vi "NR set BandWidth.vi"(8 "error in (no error)":errorcluster caption="에러 입력(에러 없음)", 10 "BW (MHz)":u32, 11 "Instrument Manager 입력":refnum<class "Instrument Manager.lvclass">) -> (0 "error out":errorcluster caption="에러 출력", 3 "Instrument Manager 출력":refnum<class "Instrument Manager.lvclass">)   [LabVIEW 2023, in "Instrument Manager.lvclass"]
uses:
  Instrument Manager.lvclass
  Module/ANRITSU Call Box/Type Definition/NR Channel Bandwidth Param.ctl
  Module/ANRITSU Call Box/Type Definition/Uplink Downlink Enum.ctl
  Instrument Manager.lvclass/Instrument Manager.ctl
  Module/ANRITSU Call Box/Interface Class/Anritsu Call Box.lvclass
  Module/ANRITSU Call Box/ANRITSU Call Box.lvlib
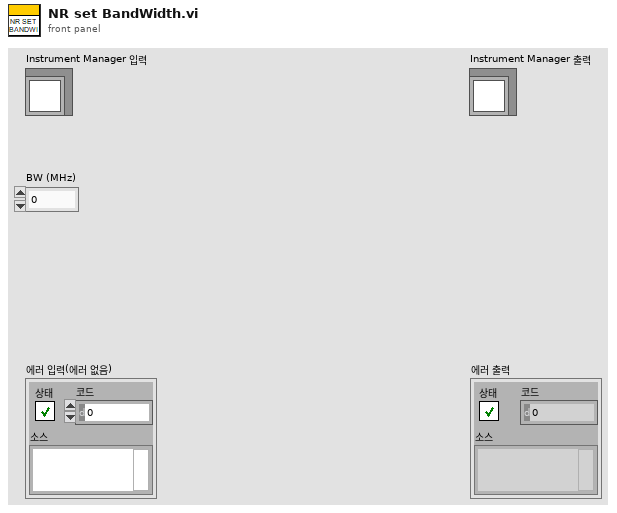
[diagram p1: front panel]
types:
  T1 = typedef "ANRITSU Call Box.lvlib/Uplink Downlink Enum.ctl" = enum16{"Uplink", "Downlink"}
  T2 = typedef "ANRITSU Call Box.lvlib/NR Channel Bandwidth Param.ctl" = cluster{"BW (MHz)":u32, "Selected CC":enum16{"PCC", "SCC", "FR2_PCC", "FR2_SCC"}, "SCC or FR2_SCC Index":u32}
  T3 = cluster{"Anritsu Call Box":refnum<class "Anritsu Call Box.lvclass">, "Spectrum Analyzer":refnum<class "Interface_Spectrum.lvclass">, "RF Switch Box":refnum<class "RF Filter Box.lvclass">, "Turn Table":refnum<class "Interface - Turn Table.lvclass">, "Mast":refnum<class "Interface - Mast.lvclass">, "3D Controller":refnum<class "Interface_3D Controller.lvclass">}
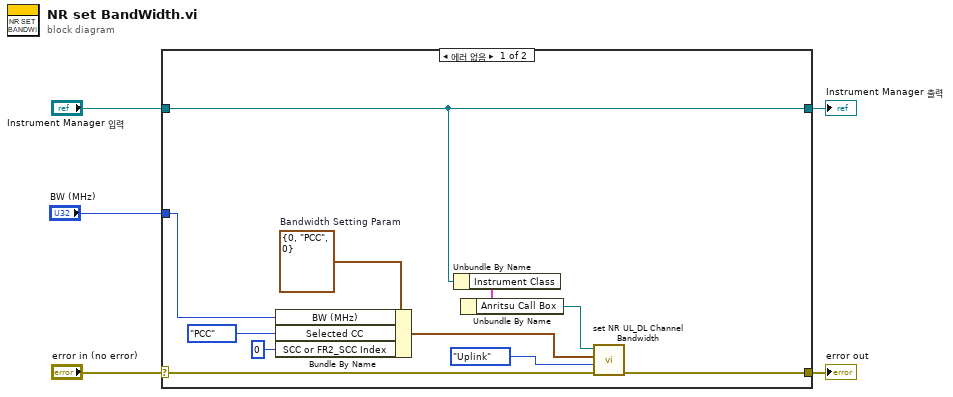
[diagram p0: block diagram]
diagram:
  n1 = case shown="에러 없음" "error in (no error)" {
    selector: "error in (no error)" -> [w11 w18]
    tunnel: [w10 w18] -> w4
    tunnel: [w9 w17] -> w2
    tunnel: "Instrument Manager 입력" -> [w9 w17]
    tunnel: "BW (MHz)" -> [w13 _]
    frame No Error {
      w16 = T2 {"BW (MHz)"=0, "Selected CC"=enum."PCC", "SCC or FR2_SCC Index"=0}  # Bandwidth Setting Param
      n2 = Bundle By Name(cluster=w16, "BW (MHz)"=w13, "Selected CC"=enum16{"PCC", "SCC", "FR2_PCC", "FR2_SCC"}."PCC", "SCC or FR2_SCC Index"=u32 0) -> (w12:T2)
      n3 = Unbundle By Name(w9) -> ("Instrument Class"=w8:T3)
      n4 = Unbundle By Name(w8) -> ("Anritsu Call Box"=w7:refnum<class "Anritsu Call Box.lvclass">)
      n5 = call-dynamic "set NR UL_DL Channel Bandwidth.vi"("error in (no error)"=w11, "Direction"=Uplink_Downlink_Enum."Uplink", "Bandwidth Setting Param"=w12, "Anritsu Call Box in"=w7) -> ("error out"=w10:errorcluster)  [unwired: 6 in, 1 out]
    }
    frame Error {
    }
  }
  "error out" <- w4
  "Instrument Manager 출력" <- w2
